vi "Check Debug.vi"(8 "error in (no error)":errorcluster, 11 "Volatus Core in":refnum<class "Volatus Core.lvclass">) -> (0 "error out":errorcluster, 3 "Volatus Core out":refnum<class "Volatus Core.lvclass">)   [LabVIEW 2020, in "Volatus.lvlib" / "Volatus Core.lvclass"]
uses:
  Volatus Core.lvclass
  C:/dev/lv20CE/relink/lv-volatus/Volatus/Module/Module.lvclass
  Module/Module.lvclass/Module.ctl
  VolatusConfig/VolatusConfigElement/VolatusConfigElement.lvclass/VolatusConfigElement.ctl
  Module/Config.vi
  VolatusConfig/VolatusConfigElement/Lookup Child by Name.vi
  VolatusConfig/VolatusConfigElement/Element.vi
  lv-cdm/CDM-Config/Config Element/Lookup Child by Name.vi
  Volatus Core.lvclass/Volatus Core.ctl
  Module/Module.lvclass
  lv-cdm/CDM-Config/Config Element/Config Element.lvclass
  C:/dev/lv20CE/relink/lv-volatus/Volatus/Volatus Core/Volatus Core.lvclass
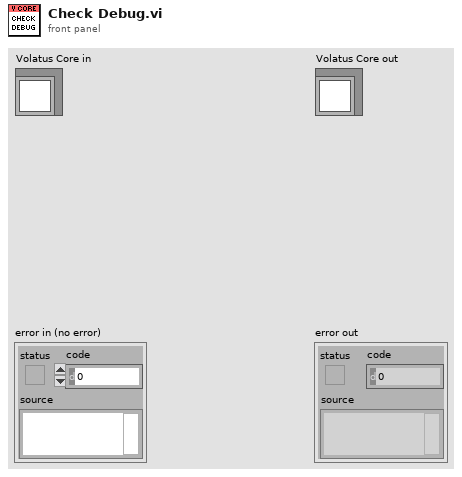
[diagram p1: front panel]
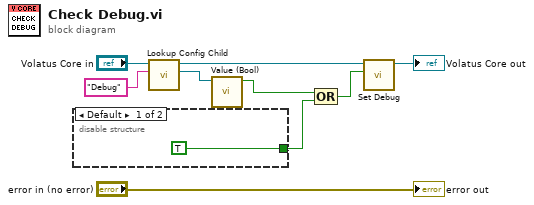
[diagram p0: block diagram]
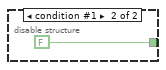
[diagram p2: hidden frame]
diagram:
  n1 = disable-structure shown="Default" {
    disable-tunnel: [TRUE FALSE] -> w1
    frame condition #0 (active) {
    }
    frame condition #1 {
    }
  }
  n2 = call "Lookup Config Child.vi"("Name"="Debug", "Module in"="Volatus Core in") -> ("Config Child"=w5:refnum<class "Config Element.lvclass">, "Module out"=w7:refnum<class "Volatus Core.lvclass">)  [unwired: 6 in, 2 out]
  n3 = call "Value (Bool).vi"("Config Element in"=w5) -> ("Bool Value"=w4:bool)  [unwired: 9 in, 1 out]
  n4 = Compound Arithmetic op=OR(w4, w1) -> (w2:bool)
  n5 = call "Set Debug.vi"("Debug"=w2, "Module in"=w7) -> ("Module out"=→"Volatus Core out":refnum<class "Volatus Core.lvclass">)  [unwired: 9 in]
  "error out" <- "error in (no error)"
